vi "Filter Strings w Pattern.vi"(10 "Exclude pattern(s) (^_)":string, 11 "Array in":string[](array[string])) -> (3 "Array out":string[](array[string]))   [LabVIEW 2014, in "VIHelpeksAPI.lvlib"]
doc: "::: VI Helpeks :::\nCopyright (c) 2000-2026 Konstantin Shifershteyn. All rights reserved."
uses:
  VIHelpeksAPI.lvlib
panel:
  # "*) To define several patterns, separate them with Line Feed \n(i.e. every line contains one pattern). Empty lines are ignored."
  # "VI Helpeks\nCopyright (c) 2012-2026 Konstantin Shifershteyn"
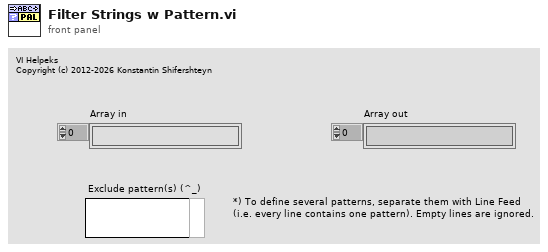
[diagram p1: front panel]
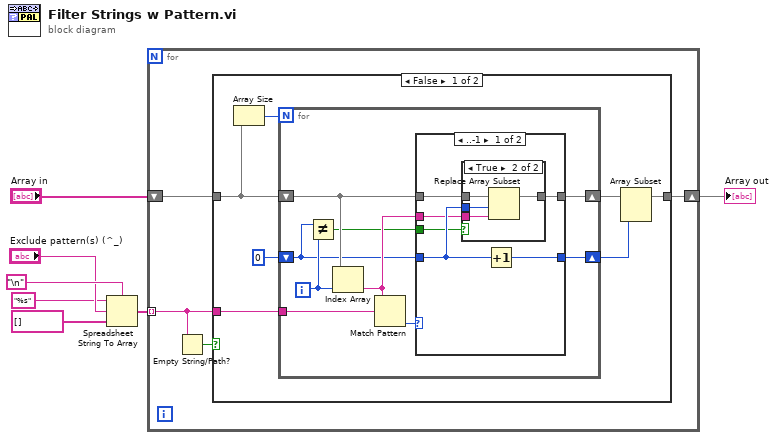
[diagram p0: block diagram]
diagram:
  n1 = Spreadsheet String To Array(delimiter (Tab)="\n", format string="%s" ("spreadsheet string"), spreadsheet string="Exclude pattern(s) (^_)", array type (2D Dbl)=string[] []) -> (array=w3:string[])
  n2 = for {
    shift-right: [w11] -> w7
    shift-left: "Array in" -> [w10]
    tunnel: w3 -> [w8] mode=indexing
    n3 = Empty String/Path?(string/path=w8) -> (empty?=w9:bool)
    n4 = case shown="False" w9 {
      tunnel: w8 -> [w17 _]
      tunnel: [w14 w41] -> w11
      tunnel: w10 -> [w12 w41]
      frame False {
        n5 = Array Size(array=w12) -> (size(s)=w13:i32)
        n6 = for {
          N: w13 -> [_]
          shift-right: [w24] -> w16
          shift-left: w12 -> [w23]
          shift-right: [w25] -> w15
          shift-left: 0 -> [w19]
          tunnel: w17 -> [w27]
          i -> [w20]
          n7 = Not Equal?(x=w19, y=w20) -> (x != y?=w21:bool)
          n8 = Index Array(array=w23, index=w20) -> (element=w22:string)
          n9 = Match Pattern(string=w22, regular expression=w27) -> (offset past match=w26:i32)  [unwired: 1 in, 3 out]
          n10 = case shown="..-1" w26 {
            tunnel: [w31 w40] -> w25
            tunnel: w19 -> [w32 w40]
            tunnel: [w30 w39] -> w24
            tunnel: w23 -> [w33 w39]
            tunnel: w22 -> [w29 _]
            tunnel: w21 -> [w28 _]
            frame ..-1 {
              n11 = case shown="True" w28 {
                tunnel: w33 -> [w34 w38]
                tunnel: w32 -> [_ w37]
                tunnel: [w34 w36] -> w30
                tunnel: w29 -> [_ w35]
                frame False {
                }
                frame True {
                  n12 = Replace Array Subset(array=w38, new element=w35, index=w37) -> (w36:string[])
                }
              }
              n13 = Increment(x=w32) -> (x+1=w31:i32)
            }
            frame 0.. {
            }
          }
        }
        n14 = Array Subset(array=w16, length=w15) -> (w14:string[])  [unwired: 1 in]
      }
      frame True {
      }
    }
  }
  "Array out" <- w7
